vi "Create Type Definition.vi"(8 "error in (no error)":errorcluster, 11 "application":refnum<vi>) -> (0 "error out":errorcluster, 3 "TypeDef VI out":refnum<vi>)   [LabVIEW 2019, in "gRPC Template Creation Utility.lvlib"]
uses:
  gRPC Template Creation Utility.lvlib
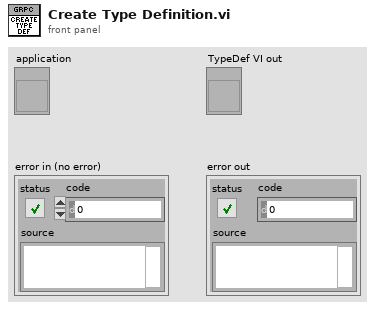
[diagram p1: front panel]
types:
  T1 = enum32{"not a control VI", "control", "typedef", "strict typedef"}
  T2 = enum32{"invalid VI type", "Standard VI", "Control VI", "Global VI", "Polymorphic VI", "Configuration VI", "SubSystem", "Facade VI", "Method VI", "Statechart Diagram VI"}
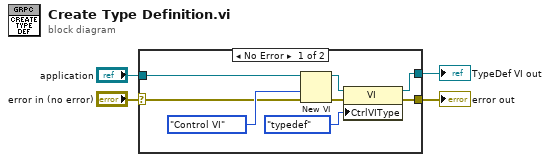
[diagram p0: block diagram]
diagram:
  n1 = case shown="No Error" "error in (no error)" {
    selector: "error in (no error)" -> [w6 w13]
    tunnel: [w12 w13] -> w4
    tunnel: [w11 _] -> w3
    tunnel: "application" -> [w5 _]
    frame No Error {
      n2 = New VI(8:w6, 9:T2."Control VI" ("vi type (standard vi)"), 11:w5) -> (0:w9:errorcluster, 3:w10:refnum<vi>)  [unwired: 4 in]
      n3 = property class="VI"(reference=w10, error in=w9, "CtrlVIType"=T1."typedef" ("Control VI Type")) -> (reference out=w11:refnum<vi>, error out=w12:errorcluster)
    }
    frame Error {
    }
  }
  "error out" <- w4
  "TypeDef VI out" <- w3
